vi "set Span Manual.vi"(8 "error in (no error)":errorcluster, 10 "Span (Hz)":dbl, 11 "FSV-40N in":refnum<class "FSV-40N.lvclass">) -> (0 "error out":errorcluster, 3 "FSV-40N out":refnum<class "FSV-40N.lvclass">)   [LabVIEW 2023, in "Spectrum Analyzer.lvlib" / "FSV-40N.lvclass"]
uses:
  FSV-40N.lvclass
  FSV-40N.lvclass/FSV-40N.ctl
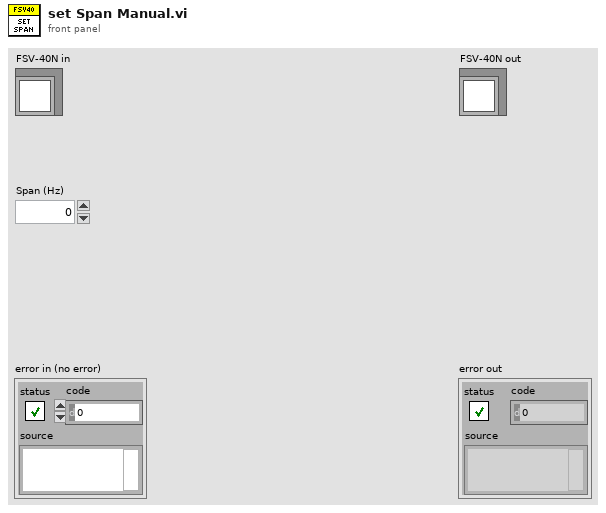
[diagram p1: front panel]
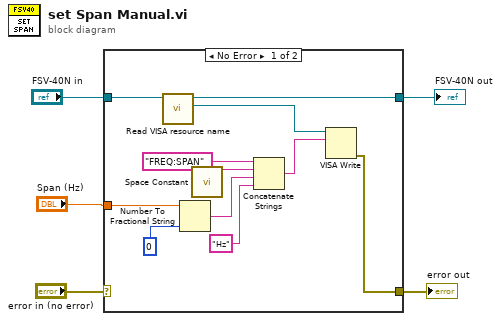
[diagram p0: block diagram]
diagram:
  n1 = case shown="No Error" "error in (no error)" {
    selector: "error in (no error)" -> [_ w17]
    tunnel: "FSV-40N in" -> [w16 w18]
    tunnel: [w7 w18] -> w4
    tunnel: [w6 w17] -> w2
    tunnel: "Span (Hz)" -> [w15 _]
    frame No Error {
      n2 = call "Read VISA resource name.vi"("FSV-40N in"=w16) -> ("VISA resource name"=w9:refnum<visa-resource-name>, "FSV-40N out"=w7:refnum<class "FSV-40N.lvclass">)  [unwired: 8 in, 1 out]
      n3 = Number To Fractional String(number=w15, precision (6)=i16 0) -> (F-format string=w11:string)  [unwired: 2 in]
      n4 = call <vilib>:"Space Constant.vi"() -> ("String"=w12:string)
      n5 = Concatenate Strings("FREQ:SPAN" ("string"), w12, w11, "Hz" ("string")) -> (w8:string)
      n6 = VISA Write(VISA resource name=w9, write buffer=w8) -> (error out=w6:errorcluster)  [unwired: 1 in, 2 out]
    }
    frame Error {
    }
  }
  "error out" <- w2
  "FSV-40N out" <- w4
